vi "RDC-water-generate_perm.vi"(8 "Increment f (10MHz)":dbl=10000000.0, 9 "Stop f (6GHz) 2":dbl=6000000000.0, 10 "Start f (300MHz)":dbl=300000000.0, 11 "water Temp (25C) [10-40C]":dbl=25.0) -> (0 "used temp":dbl, 1 "Complex Perm":cluster{dbl[], cdb[]}, 2 "Imag Perm":cluster{dbl[], dbl[]}, 3 "Real Perm":cluster{dbl[], dbl[]}, 4 "Complex perm":cdb[](array[numeric]))   [LabVIEW 2020, in "RDC-Reflection_Data_Computation.lvlib"]
doc: "Generates the water model permittivity over a frequency range (start, stop, increment) at the given water temperature (10-40 C). Returns the complex, real and imaginary permittivity and the temperature used."
uses:
  RDC-Reflection_Data_Computation.lvlib
  RDC-water-param.ctl
panel:
  out "value":T1={"temp Cx10"=25, "eps s"=78.36, "eps infi"=5.2, "tau"=8.27e-12, "eps s diff"=78.36, "eps infi diff"=5.2, "tau diff"=8.27e-12}
  out "unsigned 16bit integer":i32
  out "loss":cluster{dbl[], dbl[]}(graph)
  out "perm":cluster{dbl[], dbl[]}(graph)
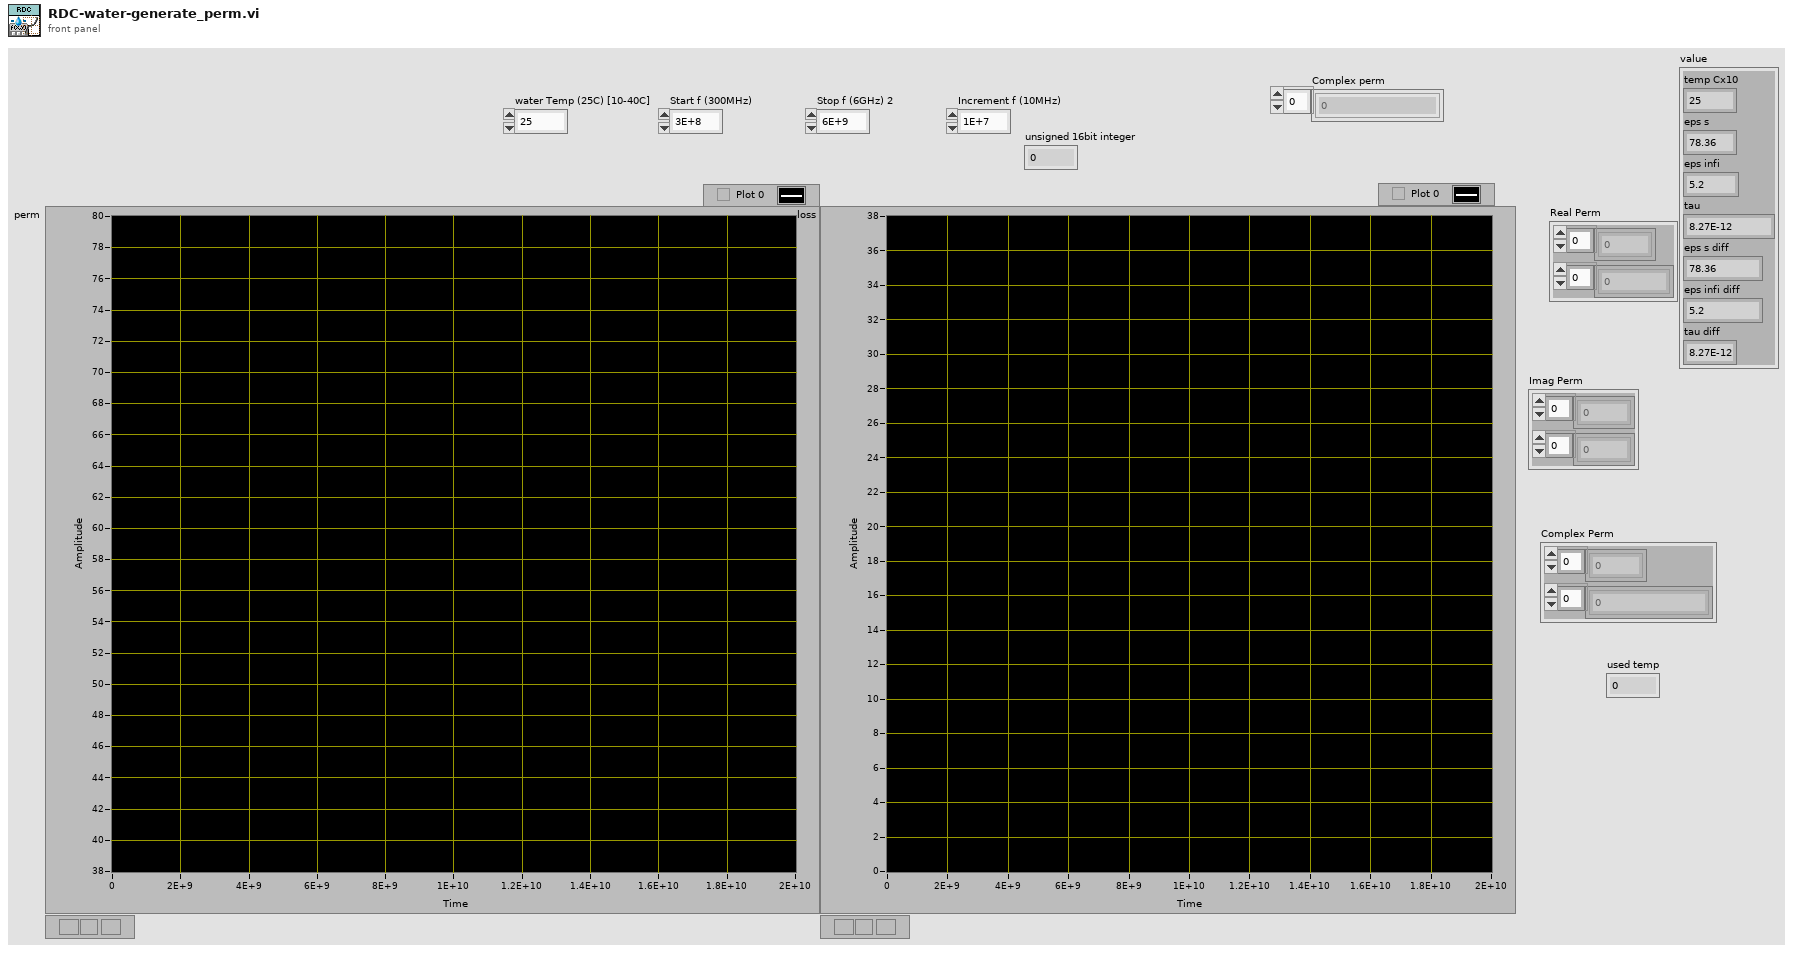
[diagram p1: front panel]
types:
  T1 = typedef "RDC-Reflection_Data_Computation.lvlib/RDC-water-param.ctl" = cluster{"temp Cx10":u16, "eps s":dbl, "eps infi":dbl, "tau":dbl, "eps s diff":dbl, "eps infi diff":dbl, "tau diff":dbl}
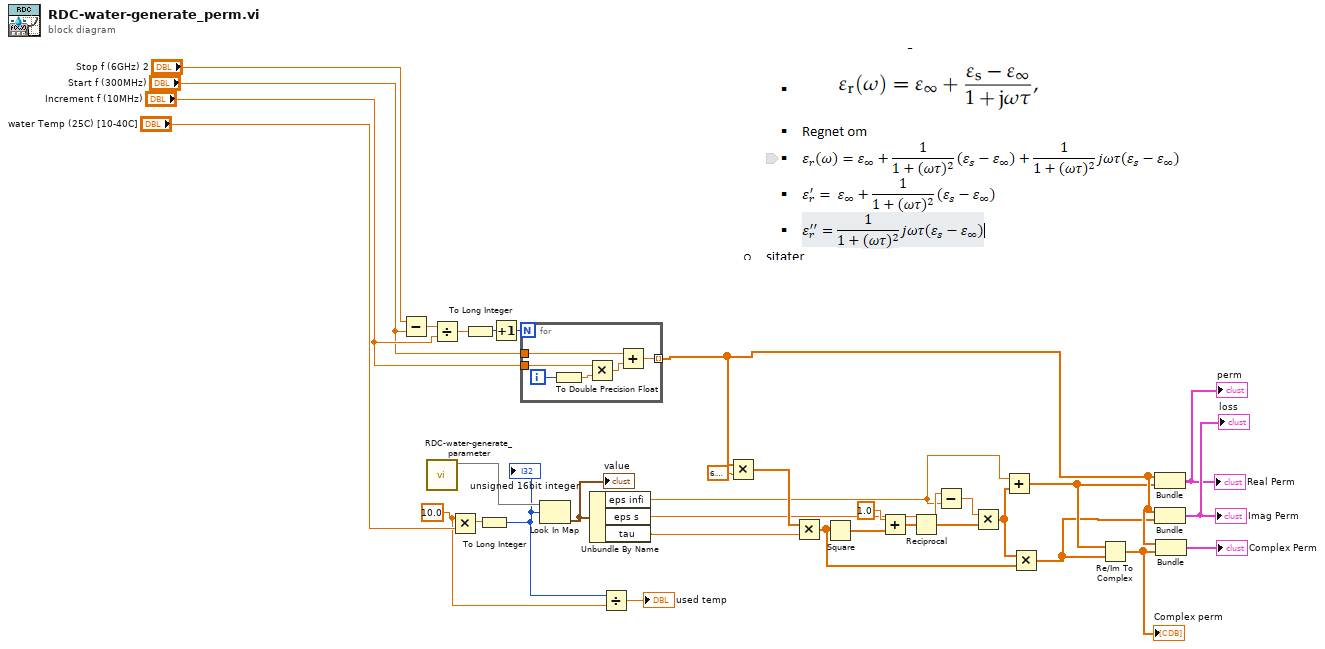
[diagram p0: block diagram]
diagram:
  w3 = 10.0 ("x")
  n1 = Subtract(x="Stop f (6GHz) 2", y="Start f (300MHz)") -> (x-y=w32:dbl)
  n2 = call "RDC-water-generate_parameter.vi"() -> ("parameter map"=w5:map{i32, T1})  [unwired: 11 in]
  n3 = Divide(x=w32, y="Increment f (10MHz)") -> (x/y=w30:dbl)
  n4 = Multiply(x=w3, y="water Temp (25C) [10-40C]") -> (x*y=w26:dbl)
  n5 = To Long Integer(number=w30) -> (32bit integer=w29:i32)
  n6 = To Long Integer(number=w26) -> (32bit integer=w4:i32)
  "unsigned 16bit integer" <- w4
  n7 = Increment(x=w29) -> (x+1=w1:i32)
  n8 = for {
    N: w1 -> [_]
    tunnel: "Start f (300MHz)" -> [w37]
    tunnel: "Increment f (10MHz)" -> [w36]
    tunnel: [w34] -> w15 mode=indexing
    i -> [w35]
    n9 = To Double Precision Float(number=w35) -> (double precision float=w39:dbl)
    n10 = Multiply(x=w36, y=w39) -> (x*y=w38:dbl)
    n11 = Add(x=w37, y=w38) -> (x+y=w34:dbl)
  }
  n12 = Look In Map(map=w5, key=w4) -> (value=w24:T1)  [unwired: 1 in, 1 out]
  "value" <- w24
  n13 = Unbundle By Name(w24) -> ("eps infi"=w13:dbl, "eps s"=w14:dbl, "tau"=w11:dbl)
  n14 = Divide(x=w4, y=w3) -> (x/y=→"used temp":dbl)
  n15 = Multiply(x=w15, y=6.283185307179586) -> (x*y=w20:dbl[])
  n16 = Multiply(x=w20, y=w11) -> (x*y=w16:dbl[])
  n17 = Square(x=w16) -> (x^2=w23:dbl[])
  n18 = Add(x=1.0, y=w23) -> (x+y=w19:dbl[])
  n19 = Reciprocal(x=w19) -> (1/x=w18:dbl[])
  n20 = Subtract(x=w14, y=w13) -> (x-y=w12:dbl)
  n21 = Multiply(x=w12, y=w18) -> (x*y=w17:dbl[])
  n22 = Add(x=w13, y=w17) -> (x+y=w10:dbl[])
  n23 = Multiply(x=w17, y=w16) -> (x*y=w9:dbl[])
  n24 = Re/Im To Complex(1:w9, 2:w10) -> (0:w28:cdb[])
  "Complex perm" <- w28
  n25 = Bundle(w15, w10) -> (→"Real Perm" →"perm":cluster{dbl[], dbl[]})  [unwired: 1 in]
  n26 = Bundle(w15, w9) -> (→"Imag Perm" →"loss":cluster{dbl[], dbl[]})  [unwired: 1 in]
  n27 = Bundle(w15, w28) -> (→"Complex Perm":cluster{dbl[], cdb[]})  [unwired: 1 in]
